vi "Check Action.vi"(6 "HRS Time":dbl, 7 "Values In":dbl[](array[numeric]), 8 "error in (no error)":errorcluster, 11 "Valve in":refnum<class "TimedPWMControl.lvclass">) -> (0 "error out":errorcluster, 2 "Actions":T1[](array[typedef]), 3 "Valve out":refnum<class "TimedPWMControl.lvclass">, 5 "Values":dbl[](array[numeric]))   [LabVIEW 2020, in "VolatusControl.lvlib" / "TimedPWMControl.lvclass"]
uses:
  TimedPWMControl.lvclass
  Control Action.ctl
  TimedPWMControl.lvclass/TimedPWMControl.ctl
  State.ctl
  Volatus/MessageQ/MessageQ.lvclass
  VolatusControl.lvlib
  lv-control/IG PID/PID/PID.lvclass
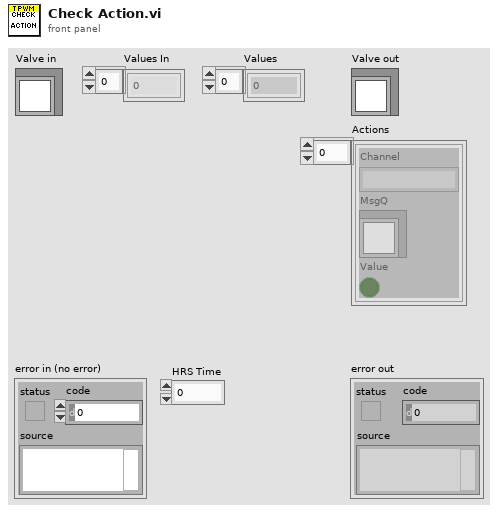
[diagram p1: front panel]
types:
  T1 = typedef "VolatusControl.lvlib/Control Action.ctl" = cluster{"Channel":string, "MsgQ":refnum<class "MessageQ.lvclass">, "Value":bool}
  T2 = typedef "VolatusControl.lvlib/TimedPWMControl.lvclass/State.ctl" = enum16{"Idle", "Start", "Enabled", "Disable"}
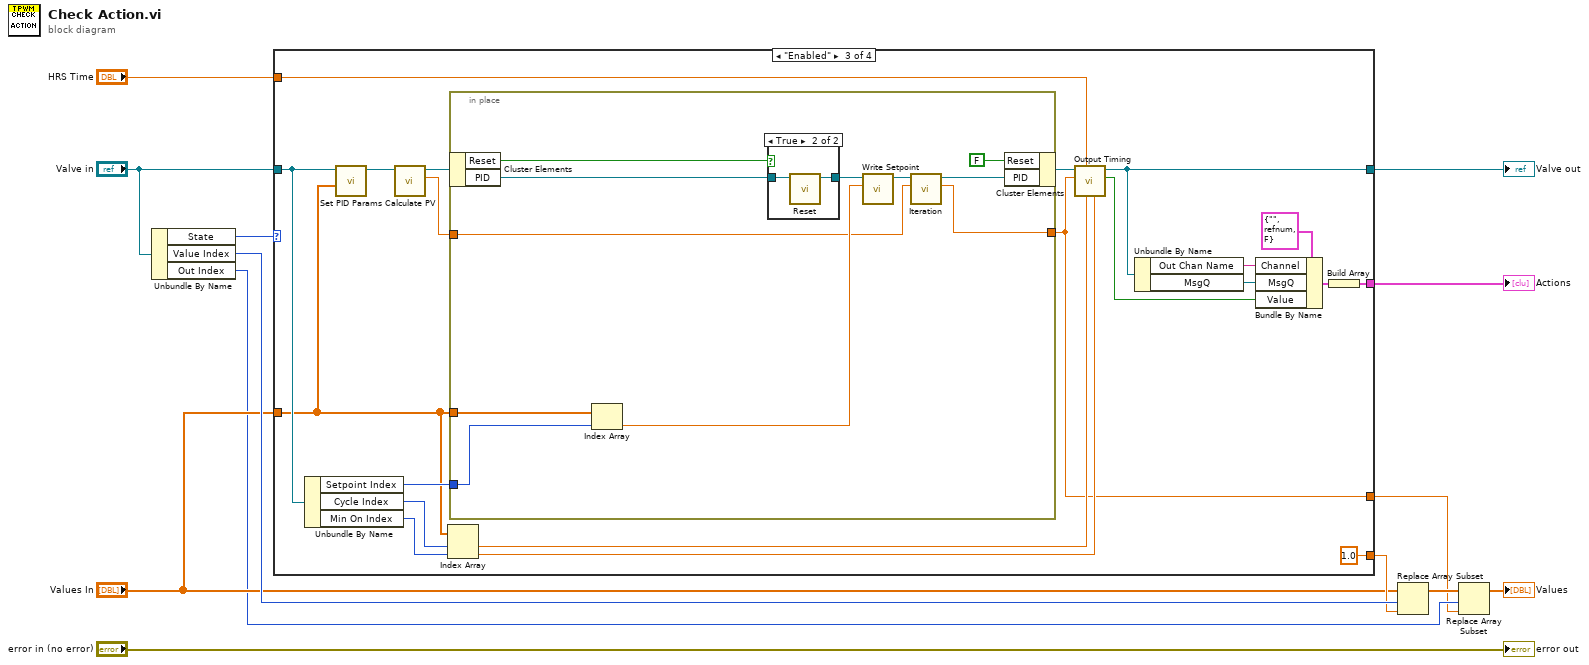
[diagram p0: block diagram]
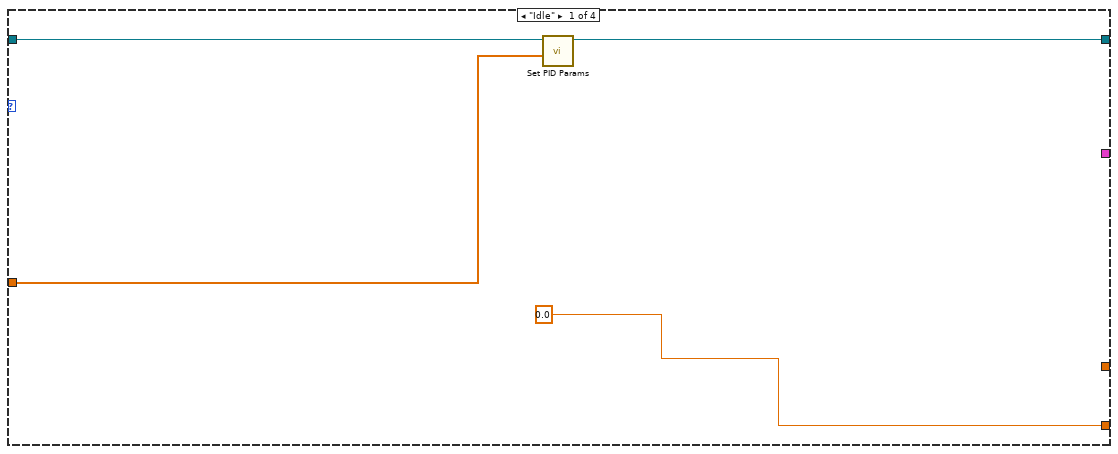
[diagram p2: hidden frame]
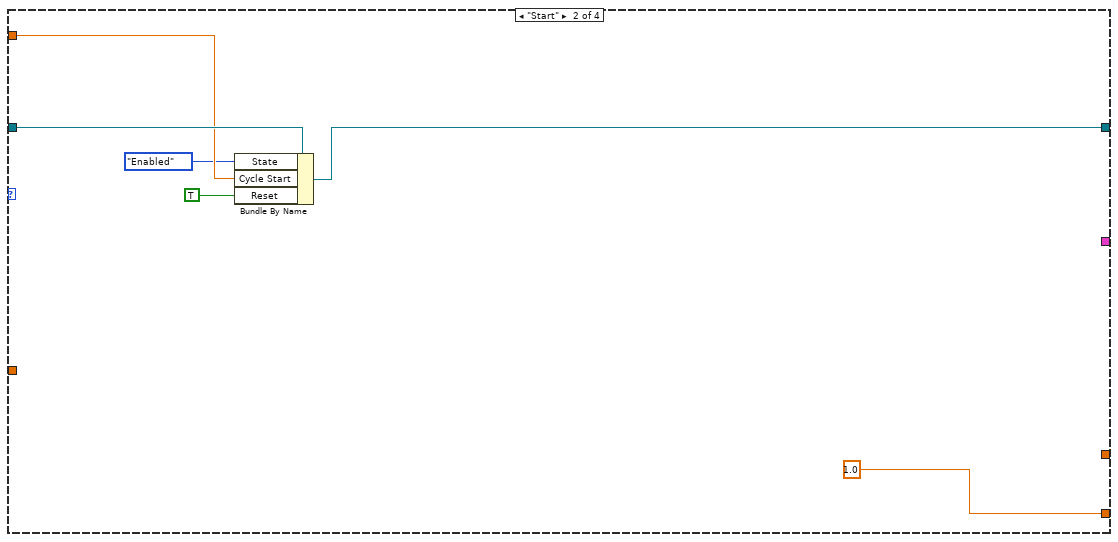
[diagram p3: hidden frame]
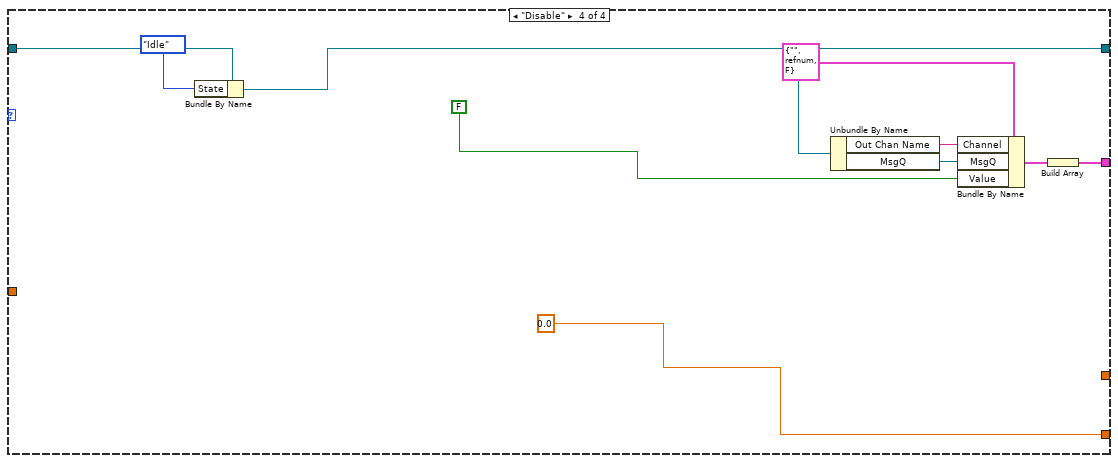
[diagram p5: hidden frame]
diagram:
  n1 = Unbundle By Name("Valve in") -> ("State"=w11:T2, "Value Index"=w12:i32, "Out Index"=w5:i32)
  n2 = case shown="\"Enabled\"" w11 {
    tunnel: [0.0 1.0 1.0 0.0] -> w10
    tunnel: [_ _ w24 w59] -> w9
    tunnel: [w15 w20 w34 w61] -> w8
    tunnel: "Values In" -> [w14 _ w27 _]
    tunnel: [_ _ w31 _] -> w3
    tunnel: "HRS Time" -> [_ w22 w30 _]
    tunnel: "Valve in" -> [w16 w23 w29 w64]
    frame "Idle" {
      n3 = call "Set PID Params.vi"("Values"=w14, "TimedPWMControl in"=w16) -> ("TimedPWMControl out"=w15:refnum<class "TimedPWMControl.lvclass">)  [unwired: 8 in, 1 out]
    }
    frame "Start" {
      n4 = Bundle By Name(cluster=w23, "State"=State."Enabled", "Cycle Start"=w22, "Reset"=TRUE) -> (w20:refnum<class "TimedPWMControl.lvclass">)
    }
    frame "Enabled" {
      n5 = Unbundle By Name(w29) -> ("Setpoint Index"=w41:i32, "Cycle Index"=w39:i32, "Min On Index"=w38:i32)
      n6 = call "Set PID Params.vi"("Values"=w27, "TimedPWMControl in"=w29) -> ("TimedPWMControl out"=w28:refnum<class "TimedPWMControl.lvclass">)  [unwired: 8 in, 1 out]
      n7 = call "Calculate PV.vi"("TimedPWMControl in"=w28) -> ("PV"=w25:dbl, "TimedPWMControl out"=w26:refnum<class "TimedPWMControl.lvclass">)  [unwired: 8 in, 1 out]
      n8 = Index Array(array=w27, index #1=w39, index #2=w38) -> (element #1=w37:dbl, element #2=w36:dbl)
      n9 = in-place {
        in-place-border: w41 -> [w53]
        in-place-border: w27 -> [w54]
        in-place-border: [w50] -> w31
        in-place-border: w25 -> [w45]
        n10 = in-place-cluster #1(w26) -> ("Reset"=w47:bool, "PID"=w46:refnum<class "PID.lvclass">)
        n11 = Index Array(array=w54, index=w53) -> (element=w52:dbl)
        n12 = case shown="True" w47 {
          tunnel: w46 -> [w56 w58]
          tunnel: [w56 w57] -> w48
          frame False {
          }
          frame True {
            n13 = call "Reset.vi"("PID in"=w58) -> ("PID out"=w57:refnum<class "PID.lvclass">)  [unwired: 9 in, 1 out]
          }
        }
        n14 = call "Write Setpoint.vi"("Setpoint"=w52, "PID in"=w48) -> ("PID out"=w55:refnum<class "PID.lvclass">)  [unwired: 8 in, 1 out]
        n15 = call "Iteration.vi"("Process Value"=w45, "PID in"=w55) -> ("Output"=w50:dbl, "PID out"=w51:refnum<class "PID.lvclass">)  [unwired: 6 in, 2 out]
        n16 = in-place-cluster #1("Reset"=FALSE, "PID"=w51) -> (w42:refnum<class "TimedPWMControl.lvclass">)
      }
      n17 = call "Output Timing.vi"("Min On"=w36, "Cycle"=w37, "HRS Time"=w30, "Out 0-1"=w31, "TimedPWMControl in"=w42) -> ("Output"=w35:bool, "TimedPWMControl out"=w34:refnum<class "TimedPWMControl.lvclass">)  [unwired: 4 in, 1 out]
      n18 = Unbundle By Name(w34) -> ("Out Chan Name"=w33:string, "MsgQ"=w32:refnum<class "MessageQ.lvclass">)
      n19 = Bundle By Name(cluster=T1 {"Channel"="", "MsgQ"=refnum, "Value"=FALSE} ("Action"), "Channel"=w33, "MsgQ"=w32, "Value"=w35) -> (w40:T1)
      n20 = Build Array(w40) -> (w24:T1[])
    }
    frame "Disable" {
      n21 = Bundle By Name(cluster=w64, "State"=State."Idle") -> (w61:refnum<class "TimedPWMControl.lvclass">)
      n22 = Unbundle By Name(w61) -> ("Out Chan Name"=w62:string, "MsgQ"=w63:refnum<class "MessageQ.lvclass">)
      n23 = Bundle By Name(cluster=T1 {"Channel"="", "MsgQ"=refnum, "Value"=FALSE} ("Action"), "Channel"=w62, "MsgQ"=w63, "Value"=FALSE) -> (w66:T1)
      n24 = Build Array(w66) -> (w59:T1[])
    }
  }
  "Valve out" <- w8
  "Actions" <- w9
  n25 = Replace Array Subset(array="Values In", new element=w10, index=w12) -> (w6:dbl[])
  n26 = Replace Array Subset(array=w6, new element=w3, index=w5) -> (→"Values":dbl[])
  "error out" <- "error in (no error)"
